vi "Start TCP Comms.vi"(8 "error in (no error)":errorcluster, 11 "Guardian in":refnum<class "Guardian.lvclass">) -> (0 "error out":errorcluster, 3 "Guardian out":refnum<class "Guardian.lvclass">)   [LabVIEW 2020, in "TALOS.lvlib" / "Guardian.lvlib" / "Guardian.lvclass"]
uses:
  Guardian.lvclass
  C:/LabVIEW Code/TALOS/builds/Actor Framework PPL/Actor Framework.lvlibp/1abvi3w/vi.lib/ActorFramework/Actor/Actor.lvclass
  C:/LabVIEW Code/TALOS/talos/Ancestor/Ancestor/Ancestor.lvclass
  Ancestor/Ancestor/Ancestor.lvclass/Ancestor.ctl
  Guardian Messages/Launch uService Msg/Launch uService Msg.lvclass/Launch uService Msg.ctl
  Guardian.lvclass/Guardian.ctl
  Guardian Messages/Message to uService Msg/Message to uService Msg.lvclass/Message to uService Msg.ctl
  Ancestor/Ancestor/Read ID.vi
  Support VIs/Generate Error.vi
  FGV/Error Memory/Get Error Description.vi
  Support VIs/Get PC name.vi
  Support VIs/Get Class Name.vi
  <vilib>/Utility/error.llb/Clear Errors.vi
  FGV/Error Memory/Error Memory Core.vi
  <vilib>/AdvancedString/Delimited String to 1D String Array.vi
  Support VIs/Circus Root Path.vi
  FGV/Error Memory/Error Crt Lvl checker.vi
  FGV/Error Memory/Error Memory Core.vi/40c8088d-b597-4017-91af-faa98e00292e.vi
  FGV/Error Memory/Error Memory Core.vi/d4a3ab98-063c-4e44-b43d-fbdcfe6c2be2.vi
  Support VIs/Global Constants.vi
  Support VIs/Global Memory.vi
  <vilib>/Utility/LVClass/Get LV Class Name.vi
  Support VIs/Is in Packed Library.vi
  Support VIs/TALOS Root path.vi
  Support VIs/Read CSV worksheet.vi
  <vilib>/Utility/error.llb/General Error Handler.vi
  <vilib>/Utility/config.llb/Open Config Data.vi
  <vilib>/Utility/config.llb/Get Section Names.vi
  <vilib>/Utility/config.llb/Get Key Names.vi
  <vilib>/Utility/config.llb/Read Key.vi
  <vilib>/Utility/config.llb/Read Key (String).vi
  <vilib>/Utility/config.llb/Close Config Data.vi
  builds/Actor Framework PPL/Actor Framework.lvlibp/1abvi3w/vi.lib/ActorFramework/Message Enqueuer/Enqueue.vi
  Support VIs/Error Log.vi
  Ancestor/Ancestor/Ancestor.lvclass
  <vilib>/Comparison/Equal/Equal Functor/Equal Functor.lvclass
  Guardian Messages/Launch uService Msg/Launch uService Msg.lvclass
  Guardian Messages/Message to uService Msg/Message to uService Msg.lvclass
  Classes/Guardian List/Guardian List.lvclass
  builds/Actor Framework PPL/Actor Framework.lvlibp/1abvi3w/vi.lib/ActorFramework/Actor/Actor.lvclass
  TALOS.lvlib
  C:/LabVIEW Code/TALOS/talos/Guardian/Guardian/Guardian.lvclass
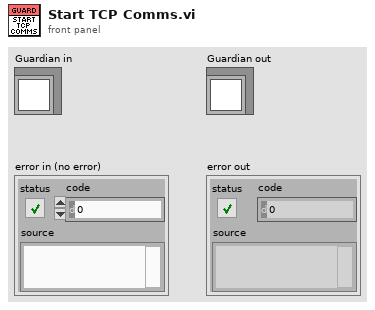
[diagram p1: front panel]
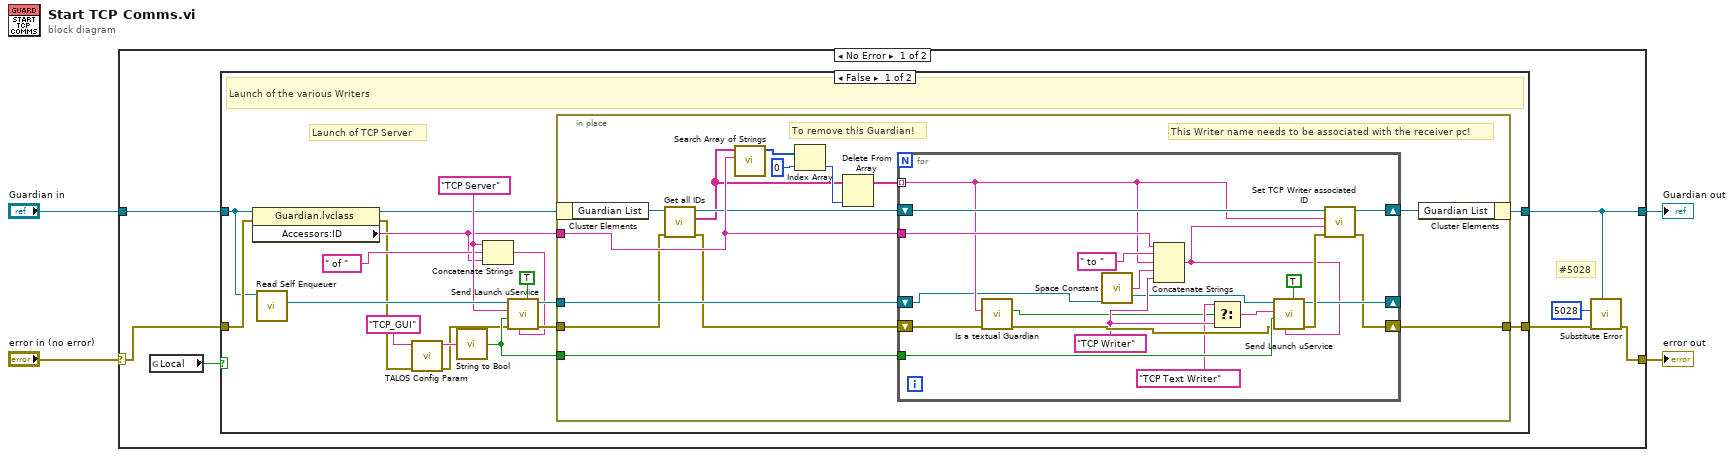
[diagram p0: block diagram]
diagram:
  n1 = case shown="No Error" "error in (no error)" {
    selector: "error in (no error)" -> [w9 w65]
    tunnel: [w7 w65] -> w4
    tunnel: "Guardian in" -> [w10 w66]
    tunnel: [w5 w66] -> w1
    frame No Error {
      # "#5028"
      n2 = global read "Global Constants.vi" "Local"() -> (w11:bool)
      n3 = case shown="False" w11 {
        tunnel: [w29 w63] -> w8
        tunnel: [w28 w64] -> w5
        tunnel: w10 -> [w23 w64]
        tunnel: w9 -> [w24 w63]
        frame False {
          w26 = "TCP Server" ("uService Class Name")
          # "Launch of TCP Server"
          # "Launch of the various Writers"
          n4 = property class="Guardian.lvclass"(reference=w23, error in=w24) -> (reference out=w22:refnum<class "Guardian.lvclass">, error out=w13:errorcluster, "Accessors:ID"=w21:string)
          n5 = call "Read Self Enqueuer.vi"("Actor"=w23) -> ("Self Enqueuer"=w27:refnum<class "Message Enqueuer.lvclass">)  [unwired: 10 in]
          n6 = call "TALOS Config Param.vi"("error in (no error)"=w13, "Parameter Name"="TCP_GUI") -> ("error out"=w12:errorcluster, "Output"=w16:string)  [unwired: 8 in]
          n7 = call "String to Bool.vi"("String"=w16) -> ("Boolean"=w14:bool)
          n8 = Concatenate Strings(w26, " of " ("string"), w21) -> (w18:string)
          n9 = call "Send Launch uService.vi"("Highlander?"=TRUE, "uService ID"=w18, "error in (no error)"=w12, "GUI?"=w14, "uService Class Name"=w26, "Message Enqueuer"=w27) -> ("error out"=w20:errorcluster, "Message Enqueuer out"=w19:refnum<class "Message Enqueuer.lvclass">)  [unwired: 4 in]
          n10 = in-place {
            in-place-border: w19 -> [w43]
            in-place-border: [w42] -> w29
            in-place-border: w20 -> [w32]
            in-place-border: w21 -> [w37]
            in-place-border: w14 -> [w30]
            # "This Writer name needs to be associated with the receiver pc!"
            # "To remove this Guardian!"
            n11 = in-place-cluster #1(w22) -> ("Guardian List"=w35:refnum<class "Guardian List.lvclass">)
            n12 = call-dynamic "Get all IDs.vi"("error in (no error)"=w32, "Guardian List in"=w35) -> ("error out"=w31:errorcluster, "All IDs"=w33:string[], "Guardian List out"=w34:refnum<class "Guardian List.lvclass">)  [unwired: 7 in]
            n13 = call "Search Array of Strings.vi"("search string"=w37, "Search array"=w33) -> ("indices"=w40:i32[])  [unwired: 8 in, 1 out]
            n14 = Index Array(array=w40, index=0) -> (element=w41:i32)
            n15 = Delete From Array(array=w33, index=w41) -> (array with subset deleted=w38:string[])  [unwired: 1 in, 1 out]
            n16 = for {
              shift-right: [w54] -> w42
              shift-left: w31 -> [w52]
              tunnel: w38 -> [w46] mode=indexing
              shift-right: [w58] -> _
              shift-left: w43 -> [w45]
              tunnel: w37 -> [w50]
              shift-right: [w53] -> w36
              shift-left: w34 -> [w61]
              tunnel: w30 -> [w57]
              w48 = "TCP Writer" ("uService Class Name")
              n17 = call "Is a textual Guardian.vi"("error in (no error)"=w52, "Target GD ID"=w46) -> ("error out"=w51:errorcluster, "Textual?"=w44:bool)  [unwired: 8 in]
              n18 = call <vilib>:"Space Constant.vi"() -> ("String"=w59:string)
              n19 = Concatenate Strings(w50, " to " ("string"), w46, w59, w48) -> (w56:string)
              n20 = Select(t="TCP Text Writer" ("uService Class Name"), s=w44, f=w48) -> (s? t:f=w49:string)
              n21 = call "Send Launch uService.vi"("Highlander?"=TRUE, "uService ID"=w56, "error in (no error)"=w51, "GUI?"=w57, "uService Class Name"=w49, "Message Enqueuer"=w45) -> ("error out"=w60:errorcluster, "Message Enqueuer out"=w58:refnum<class "Message Enqueuer.lvclass">)  [unwired: 4 in]
              n22 = call-dynamic "Set TCP Writer associated ID.vi"("error in (no error)"=w60, "TCP Writer associated ID"=w56, "ID"=w46, "Guardian List in"=w61) -> ("error out"=w54:errorcluster, "Guardian List out"=w53:refnum<class "Guardian List.lvclass">)  [unwired: 6 in]
            }
            n23 = in-place-cluster #1("Guardian List"=w36) -> (w28:refnum<class "Guardian.lvclass">)
          }
        }
        frame True {
          # "We are running in locale, no comm.s with the other computers (Kasli included)."
        }
      }
      n24 = call "Substitute Error.vi"("LabVIEW Object"=w5, "error in (no error)"=w8, "Error Code"=5028) -> ("error out"=w7:errorcluster)  [unwired: 8 in]
    }
    frame Error {
    }
  }
  "error out" <- w4
  "Guardian out" <- w1
